vi "ACW ini file Read.vi"(5 "error in (no error) 2":errorcluster, 10 "configuration file path":path) -> (12 "ACW Voltage":dbl, 14 "Ramp Time":dbl, 15 "LO SET":dbl, 16 "HI SET":dbl, 17 "Test Time":dbl, 18 "Freq":u32, 19 "error in (no error) 3":errorcluster)   [LabVIEW 2021]
uses:
  Template/Main_VI/Control/Ini.ctl
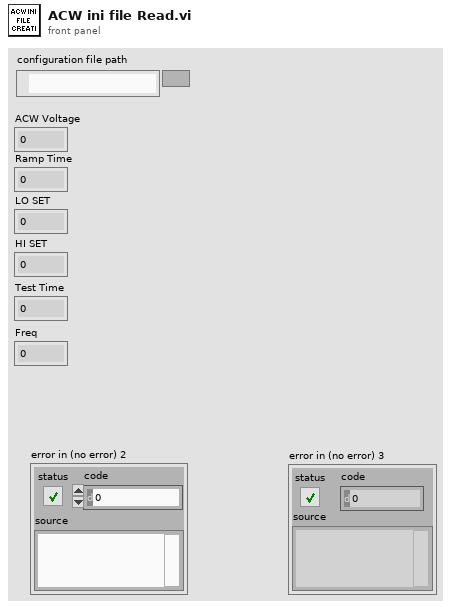
[diagram p1: front panel]
types:
  T1 = typedef "Ini.ctl" = enum16{"Write", "Read"}
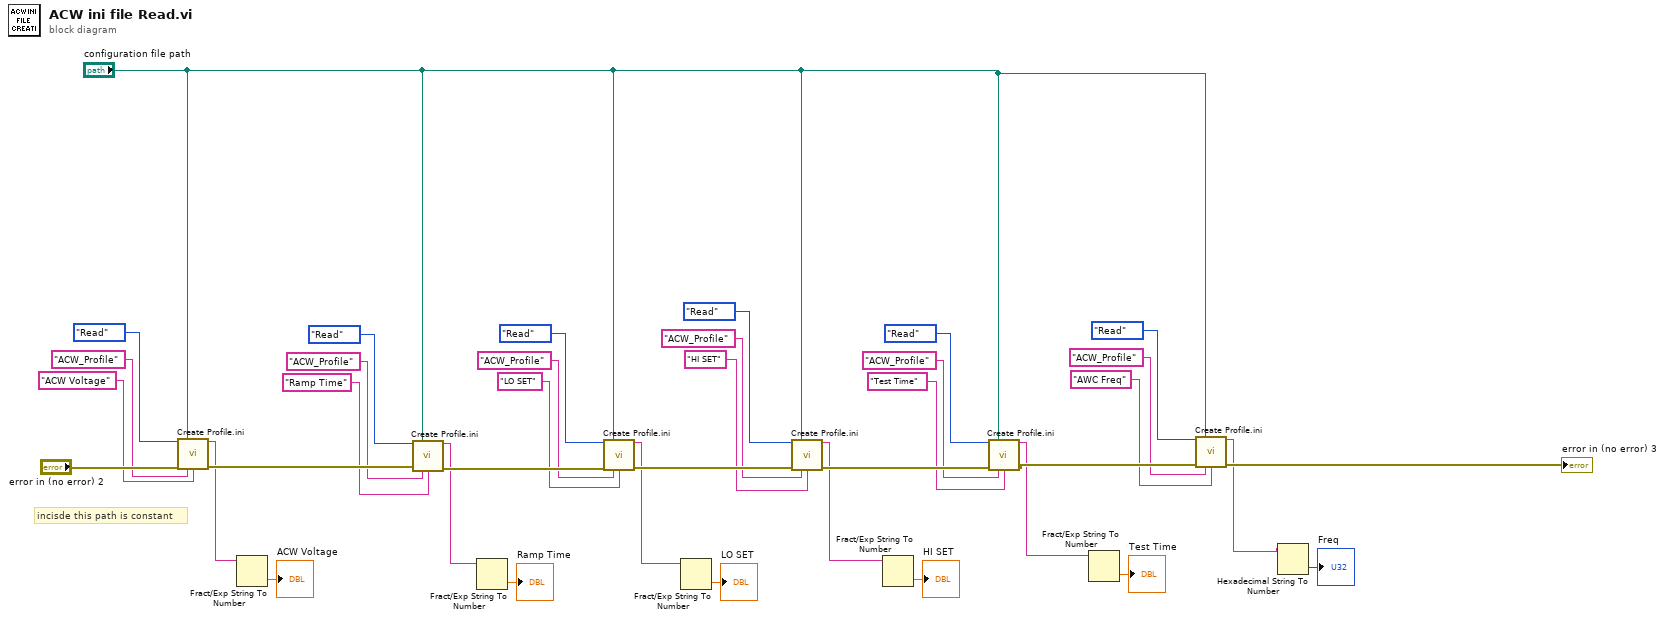
[diagram p0: block diagram]
diagram:
  # "incisde this path is constant"
  n1 = call "Create Profile.ini.vi"(0:Ini."Read", "configuration file path"="configuration file path", "error in (no error)"="error in (no error) 2", "Read Section"="ACW_Profile" ("Write Section"), "Read Key"="ACW Voltage" ("Write key")) -> ("value"=w14:string, "error in (no error) 3"=w33:errorcluster)  [unwired: 9 in]
  n2 = Fract/Exp String To Number(string=w14) -> (number=→"ACW Voltage":dbl)  [unwired: 3 in, 1 out]
  n3 = call "Create Profile.ini.vi"(0:Ini."Read", "configuration file path"="configuration file path", "error in (no error)"=w33, "Read Section"="ACW_Profile" ("Write Section"), "Read Key"="Ramp Time" ("Write key")) -> ("value"=w13:string, "error in (no error) 3"=w32:errorcluster)  [unwired: 9 in]
  n4 = Fract/Exp String To Number(string=w13) -> (number=→"Ramp Time":dbl)  [unwired: 3 in, 1 out]
  n5 = call "Create Profile.ini.vi"(0:Ini."Read", "configuration file path"="configuration file path", "error in (no error)"=w32, "Read Section"="ACW_Profile" ("Write Section"), "Read Key"="LO SET" ("Write key")) -> ("value"=w12:string, "error in (no error) 3"=w31:errorcluster)  [unwired: 9 in]
  n6 = Fract/Exp String To Number(string=w12) -> (number=→"LO SET":dbl)  [unwired: 3 in, 1 out]
  n7 = call "Create Profile.ini.vi"(0:Ini."Read", "configuration file path"="configuration file path", "error in (no error)"=w31, "Read Section"="ACW_Profile" ("Write Section"), "Read Key"="HI SET" ("Write key")) -> ("value"=w11:string, "error in (no error) 3"=w30:errorcluster)  [unwired: 9 in]
  n8 = Fract/Exp String To Number(string=w11) -> (number=→"HI SET":dbl)  [unwired: 3 in, 1 out]
  n9 = call "Create Profile.ini.vi"(0:Ini."Read", "configuration file path"="configuration file path", "error in (no error)"=w30, "Read Section"="ACW_Profile" ("Write Section"), "Read Key"="Test Time" ("Write key")) -> ("value"=w10:string, "error in (no error) 3"=w27:errorcluster)  [unwired: 9 in]
  n10 = Fract/Exp String To Number(string=w10) -> (number=→"Test Time":dbl)  [unwired: 3 in, 1 out]
  n11 = call "Create Profile.ini.vi"(0:Ini."Read", "configuration file path"="configuration file path", "error in (no error)"=w27, "Read Section"="ACW_Profile" ("Write Section"), "Read Key"="AWC Freq" ("Write key")) -> ("value"=w2:string, "error in (no error) 3"=→"error in (no error) 3":errorcluster)  [unwired: 9 in]
  n12 = Hexadecimal String To Number(string=w2) -> (number=→"Freq":u32)  [unwired: 2 in, 1 out]
